vi "DrumSeq_Pulsed_Example.vi"() -> ()   [LabVIEW 2019]
uses:
  <vilib>/Rock Robotics/WPI/ThirdParty/JAS_Junk/TrajLib/Enum/AutoHelperSequence_Step_Enum.ctl
  <vilib>/Rock Robotics/WPI/ThirdParty/JAS_Junk/TrajLib/VI/Util_GetTime_U32.vi
  <vilib>/Rock Robotics/WPI/ThirdParty/JAS_Junk/TrajLib/VI/BoolCmd_Recv_Internal.vi
  <vilib>/Rock Robotics/WPI/ThirdParty/JAS_Junk/TrajLib/Timer_New.vi
  <vilib>/Rock Robotics/WPI/ThirdParty/JAS_Junk/TrajLib/VI/BoolCmd_Send_Internal.vi
  <vilib>/Rock Robotics/WPI/ThirdParty/JAS_Junk/TrajLib/VI/BoolCmd_ObtainQueue.vi
  <vilib>/Rock Robotics/WPI/ThirdParty/JAS_Junk/TrajLib/VI/Util_GetTime_U64.vi
  <vilib>/Utility/semaphor.llb/Obtain Semaphore Reference.vi
  <vilib>/Rock Robotics/WPI/ThirdParty/JAS_Junk/TrajLib/Timer_Reset.vi
  <vilib>/Rock Robotics/WPI/ThirdParty/JAS_Junk/TrajLib/VI/Timer_Restart.vi
  <vilib>/Rock Robotics/WPI/ThirdParty/JAS_Junk/TrajLib/Timer_HasPeriodPassedOnce.vi
  <vilib>/Rock Robotics/WPI/ThirdParty/JAS_Junk/TrajLib/Trajectory_Library.lvlib
panel:
  in  "Teleop Action\nCancel":bool
  out "Auto Step Number":T1
  out "Auto\nActive":bool
  in  "Start\nAutonomous":bool
  in  "Teleop Action\nCapture":bool
  out "Hand Control \nOutput":bool
  out "Waveform Chart":cluster{i16, i16}(graph)
  out "Arm Control\nOutput":bool
  # "PULSED DRUM SEQUENCER"
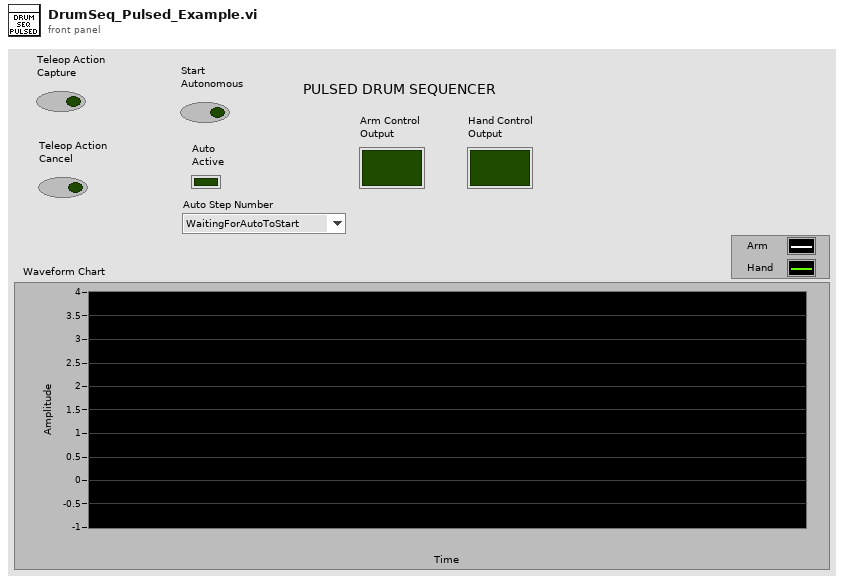
[diagram p1: front panel]
types:
  T1 = typedef "Trajectory_Library.lvlib/AutoHelperSequence_Step_Enum.ctl" = enum16{"WaitingForAutoToStart", "Step 1", "Step 2", "Step 3", "Step 4", "Step 5", "Step 6", "Step 7", "Step 8", "Step 9", "Step 10", "Step 11", "Step 12", "Step 13", "Step 14", "Step 15", "Step 16", "Step 17", "Step 18", "Step 19", "Step 20", "Step 21", "Step 22", "Step 23", "Step 24", "Step 25", "Step 26", "Step 27", "Step 28", "Step 29", "Step 30", "Step 31", "Step 32", "AutoDone"}
  T2 = typedef "Trajectory_Library.lvlib/DrumSequence_Step_Enum.ctl" = enum16{"Do Nothing", "Step 1", "Step 2", "Step 3", "Step 4", "Step 5", "Step 6", "Step 7", "Step 8", "Step 9", "Step 10", "Step 11", "Step 12", "Step 13", "Step 14", "Step 15", "Step 16", "Step 17", "Step 18", "Step 19", "Step 20", "Step 21", "Step 22", "Step 23", "Step 24", "Step 25", "Step 26", "Step 27", "Step 28", "Step 29", "Step 30", "Step 31", "Step 32", "Cancel", "Initialize", "Error"}
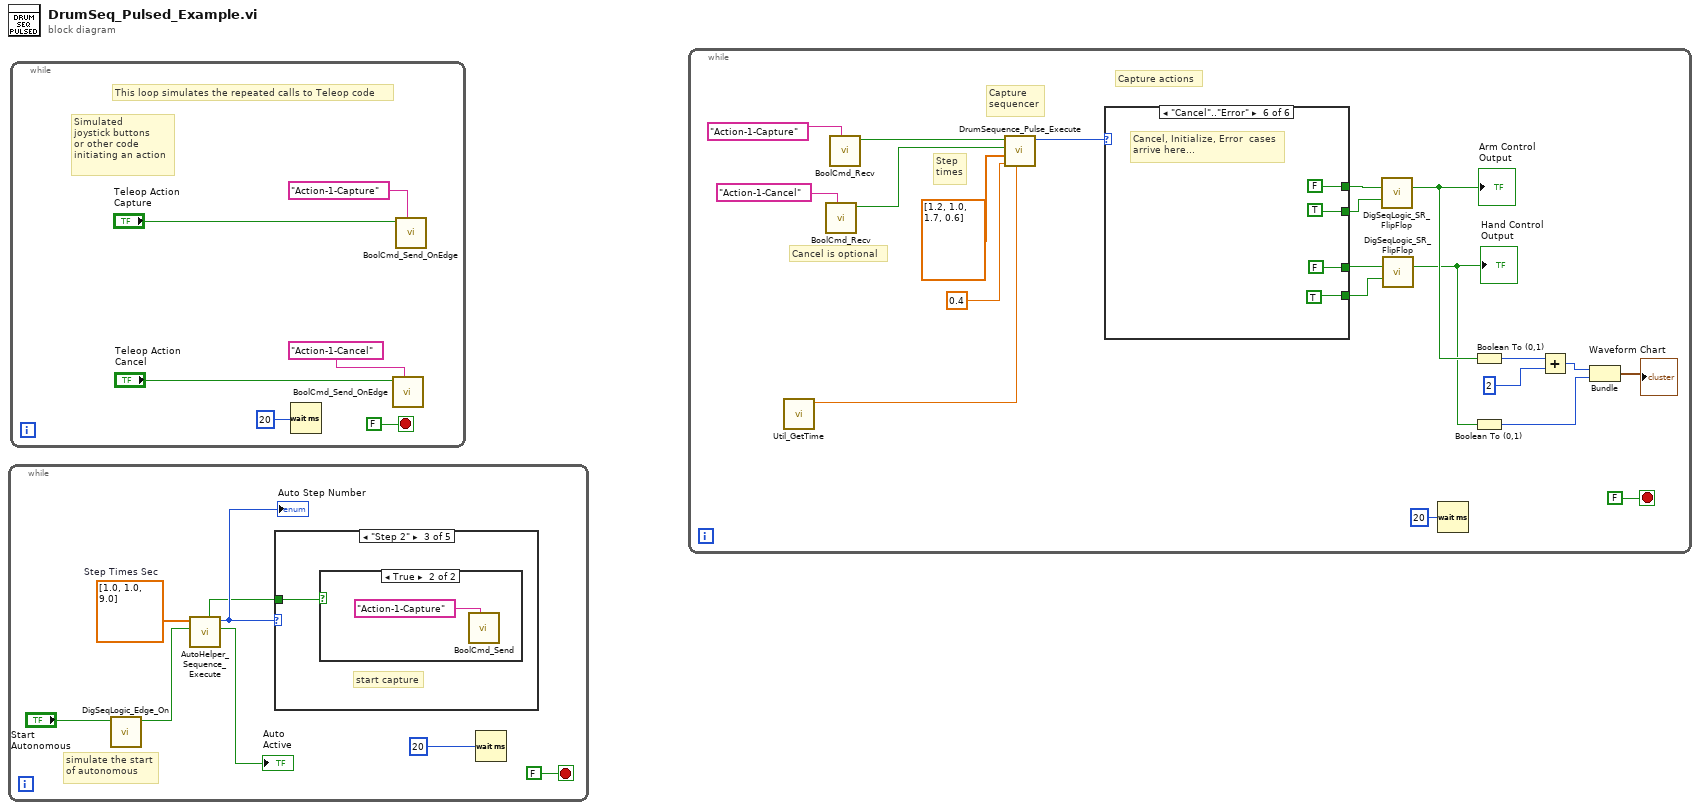
[diagram p0: block diagram]
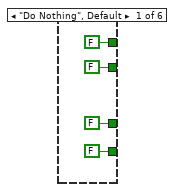
[diagram p2: hidden frame]
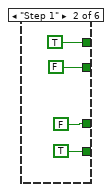
[diagram p3: hidden frame]
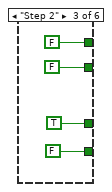
[diagram p4: hidden frame]
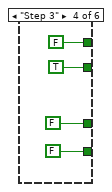
[diagram p5: hidden frame]
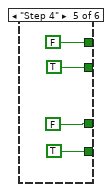
[diagram p6: hidden frame]
diagram:
  n1 = while {
    stop <- FALSE stop-if-true
    w5 = dbl[] [1.0, 1.0, 9.0]  # Step Times Sec
    # "simulate the start\nof autonomous"
    n2 = call <vilib>:"DigSeqLogic_Edge_On.vi"("Input"="Start\nAutonomous") -> ("On Edge"=w4:bool)  [unwired: 10 in]
    n3 = call <vilib>:"AutoHelper_Sequence_Execute.vi"("Initiate"=w4, "Step Times Sec"=w5) -> ("Seq  Active"=→"Auto\nActive":bool, "Step Number State"=w3:T1, "New Step"=w2:bool)  [unwired: 5 in, 2 out]
    "Auto Step Number" <- w3
    n4 = case shown="\"Step 2\"" w3 {
      tunnel: w2 -> [_ _ w9 _ _]
      frame "WaitingForAutoToStart", Default {
        # "do nothing"
      }
      frame "Step 1" {
        # "do nothing"
      }
      frame "Step 2" {
        # "start capture"
        n5 = case shown="True" w9 {
          frame False {
          }
          frame True {
            n6 = call <vilib>:"BoolCmd_Send.vi"("Command Name"="Action-1-Capture") -> ()  [unwired: 10 in, 1 out]
          }
        }
      }
      frame "Step 3" {
        # "Do nothing"
      }
      frame "AutoDone" {
        # "Auto is done."
      }
    }
    n7 = Wait (ms)(milliseconds to wait=u32 20 ("milliseconds to wait 2")) -> ()  [unwired: 1 out]
  }
  n8 = while {
    stop <- FALSE stop-if-true
    # "Simulated\njoystick buttons\nor other code \ninitiating an action"
    # "This loop simulates the repeated calls to Teleop code"
    n9 = Wait (ms)(milliseconds to wait=u32 20) -> ()  [unwired: 1 out]
    n10 = call <vilib>:"BoolCmd_Send_OnEdge.vi"("Command Name"="Action-1-Cancel", "Value"="Teleop Action\nCancel") -> ()  [unwired: 9 in, 1 out]
    n11 = call <vilib>:"BoolCmd_Send_OnEdge.vi"("Command Name"="Action-1-Capture", "Value"="Teleop Action\nCapture") -> ()  [unwired: 9 in, 1 out]
  }
  n12 = while {
    stop <- FALSE stop-if-true
    # "Step\ntimes"
    # "Cancel is optional"
    # "Capture actions"
    # "Capture\nsequencer"
    n13 = call <vilib>:"Util_GetTime.vi"() -> ("FPGA_Time_Seconds"=w31:dbl)  [unwired: 9 in, 2 out]
    n14 = call <vilib>:"BoolCmd_Recv.vi"("Command Name"="Action-1-Cancel") -> ("New Request"=w23:bool)  [unwired: 9 in, 1 out]
    n15 = call <vilib>:"BoolCmd_Recv.vi"("Command Name"="Action-1-Capture") -> ("New Request"=w24:bool)  [unwired: 9 in, 1 out]
    n16 = call <vilib>:"DrumSequence_Pulse_Execute.vi"("Pass_Through_Time"=w31, "Cancel Time Sec"=0.4, "Step Times Sec"=dbl[] [1.2, 1.0, 1.7, 0.6], "Cancel"=w23, "Initiate"=w24) -> ("Step Number State"=w32:T2)  [unwired: 3 in, 3 out]
    n17 = case shown="\"Cancel\"..\"Error\"" w32 {
      tunnel: [FALSE TRUE FALSE FALSE FALSE FALSE] -> w22
      tunnel: [FALSE FALSE TRUE FALSE FALSE FALSE] -> w20
      tunnel: [FALSE FALSE FALSE TRUE TRUE TRUE] -> w18
      tunnel: [FALSE TRUE FALSE FALSE TRUE TRUE] -> w17
      frame "Do Nothing", Default {
      }
      frame "Step 1" {
      }
      frame "Step 2" {
      }
      frame "Step 3" {
      }
      frame "Step 4" {
      }
      frame "Cancel".."Error" {
        # "Cancel, Initialize, Error  cases\narrive here..."
      }
    }
    n18 = call <vilib>:"DigSeqLogic_SR_FlipFlop.vi"("Set"=w22, "Reset"=w18) -> ("Output"=w21:bool)  [unwired: 12 in, 1 out]
    "Arm Control\nOutput" <- w21
    n19 = call <vilib>:"DigSeqLogic_SR_FlipFlop.vi"("Set"=w20, "Reset"=w17) -> ("Output"=w19:bool)  [unwired: 12 in, 1 out]
    "Hand Control \nOutput" <- w19
    n20 = Wait (ms)(milliseconds to wait=u32 20) -> ()  [unwired: 1 out]
    n21 = Boolean To (0,1)(Boolean=w21) -> (0, 1=w28:i16)
    n22 = Boolean To (0,1)(Boolean=w19) -> (0, 1=w26:i16)
    n23 = Add(x=w28, y=i16 2) -> (x+y=w27:i16)
    n24 = Bundle(w27, w26) -> (→"Waveform Chart":cluster{i16, i16})  [unwired: 1 in]
  }
